vi "channel operation tests.vi"() -> (3 "channels match":bool)   [LabVIEW 2014, in "TEC tests.lvlib"]
uses:
  TEC tests.lvlib
  configuration/TEC configuration.lvclass/TEC configuration.ctl
  configuration/Write channels.vi
  configuration/TEC configuration.lvclass
panel:
  out "error out":errorcluster
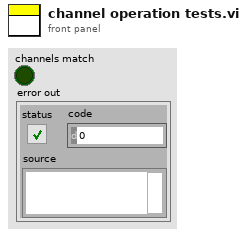
[diagram p1: front panel]
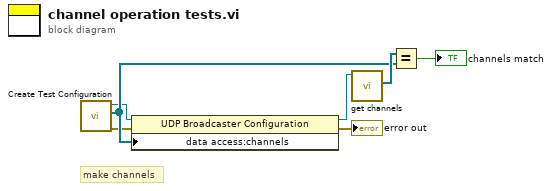
[diagram p0: block diagram]
diagram:
  # "make channels"
  n1 = call "Create Test Configuration.vi"() -> ("error out"=w2:errorcluster, "Array"=w4:refnum<class "TBM channel.lvclass">[], "TEC configuration out"=w3:refnum<class "TEC configuration.lvclass">)  [unwired: 8 in, 1 out]
  n2 = property class="UDP Broadcaster Configuration"(reference=w3, error in=w2, "data access:channels"=w4) -> (reference out=w5:refnum<class "TEC configuration.lvclass">, error out=→"error out":errorcluster)
  n3 = call-dynamic "get channels.vi"("TEC configuration in"=w5) -> ("channels"=w7:refnum<class "TBM channel.lvclass">[])  [unwired: 9 in, 1 out]
  n4 = Equal?(x=w7, y=w4) -> (x = y?=→"channels match":bool)
